vi "EndevoGOOP400Provider_Configuration.vi"(1 "ClassRef/ClassPath(If empty Configuration default will be modified)":variant, 5 "Error In":errorcluster) -> (15 "SelectedWireStyleIndex":i32, 19 "Error Out":errorcluster)   [LabVIEW 2020]
uses:
  Common/LvIcon_class/GDSLvIcon_ColorControl.ctl
  SubVIs/GOOP_WirePattern.ctl
  Common/ScriptingFunctions/Scripting_ConnectorPanePatternType.ctl
  Provider_BaseClassInterface/BaseProvider_SubVIs/BaseProvider_WireStyleType.ctl
  SubVIs/GOOP_WireConfigurationType.ctl
  Common/CommonVIs/CommonVIs_ClassIconSelection_Action.ctl
  Provider_BaseClassInterface/BaseProvider_SubVIs/BaseProvider_FileNamingOption.ctl
  GOOP400_SubVIs/GOOP400_Options.ctl
panel:
  in  "File naming option":T1(ring)
  out "IconSelection":picture
  in  "_FlatFolderStructure":bool caption="Use flat folder structure for new classes"
  in  "WireStyleList":T2[](array[typedef])
  in  "DiscardChanges":bool
  in  "Update/AddWireStyle":bool
  in  "DeleteWireStyle":bool
  in  "Down":bool
  in  "Up":bool
  in  "WireStyleName":string caption="Selected Wire Style Name"
  out "ProductPicture":picture
  out "Icon":picture
  in  "_Dice":cluster{"Boolean 2":bool, "Dice 2":bool}
  in  "_DefaultConnectorPanePattern":T3 caption="Default Connector Pane Pattern" items=["4x4x4", "5x6x5", "6x8x6"]
  in  "_HelpDefaultConfiguration":bool
  in  "_Help":bool
  out "_ClassItemIconApperance":string caption="Class Item Icon Appearance"
  out "_WireApperance":string
  in  "_SetToDefaultForAllClasses":bool caption="Set this to default\nfor all future classes"
  in  "_Cancel":bool
  out "_Preview":picture caption="Preview"
  in  "_Icon":u16(ring) caption="Icon" items=["BlueFull", "BlueFrame", "InterfaceBlue", "BlueCircle", "BrownFull", "BrownFrame", "InterfaceBrown", "BrownCircle", "BurgundyFull", "BurgundyFrame", "InterfaceBurgundy", "BurgundyCircle", "CyanFull", "CyanFrame", "InterfaceCyan", "CyanCircle", "DarkBlueFull", "DarkBlueFrame", "InterfaceDarkBlue", "DarkBlueCircle", "ForestGreenFull", "ForestGreenFrame", "InterfaceForestGreen", "ForestGreenCircle", "GrayFull", "GrayFrame", "InterfaceGray", "GrayCircle", "GreenFull", "GreenFrame", "InterfaceGreen", "GreenCircle", "LightGreenFull", "LightGreenFrame", "InterfaceLightGreen", "LightGreenCircle", "LightRedFull", "LightRedFrame", "InterfaceLightRed", "LightRedCircle", "PinkFull", "PinkFrame", "InterfacePink", "PinkCircle", "PurpleFull", "PurpleFrame", "InterfacePurple", "PurpleCircle", "RedFull", "RedFrame", "InterfaceRed", "RedCircle", "YellowFull", "YellowFrame", "InterfaceYellow", "YellowCircle"]
  in  "_TunnelsAndTerminalsColors":T4 caption="Tunnels and \nTerminals Colors"
  in  "_CenterColor2":T4 caption="Pattern Colors"
  in  "_CenterColor1":T4 caption="Pattern Colors"
  in  "_CenterPattern":T5 caption="Center pattern"
  in  "_EdgeColor":T4 caption="Edge color"
  in  "_CenterThickness":T6(ring) caption="Center thickness"
  in  "_EdgeThickness":T7(ring) caption="Edge thickness"
  out "Wire preview":picture
  in  "_Done":bool
  # "Wire Configuration"
  # "Wire Appearance"
  # "GOOP4 Options"
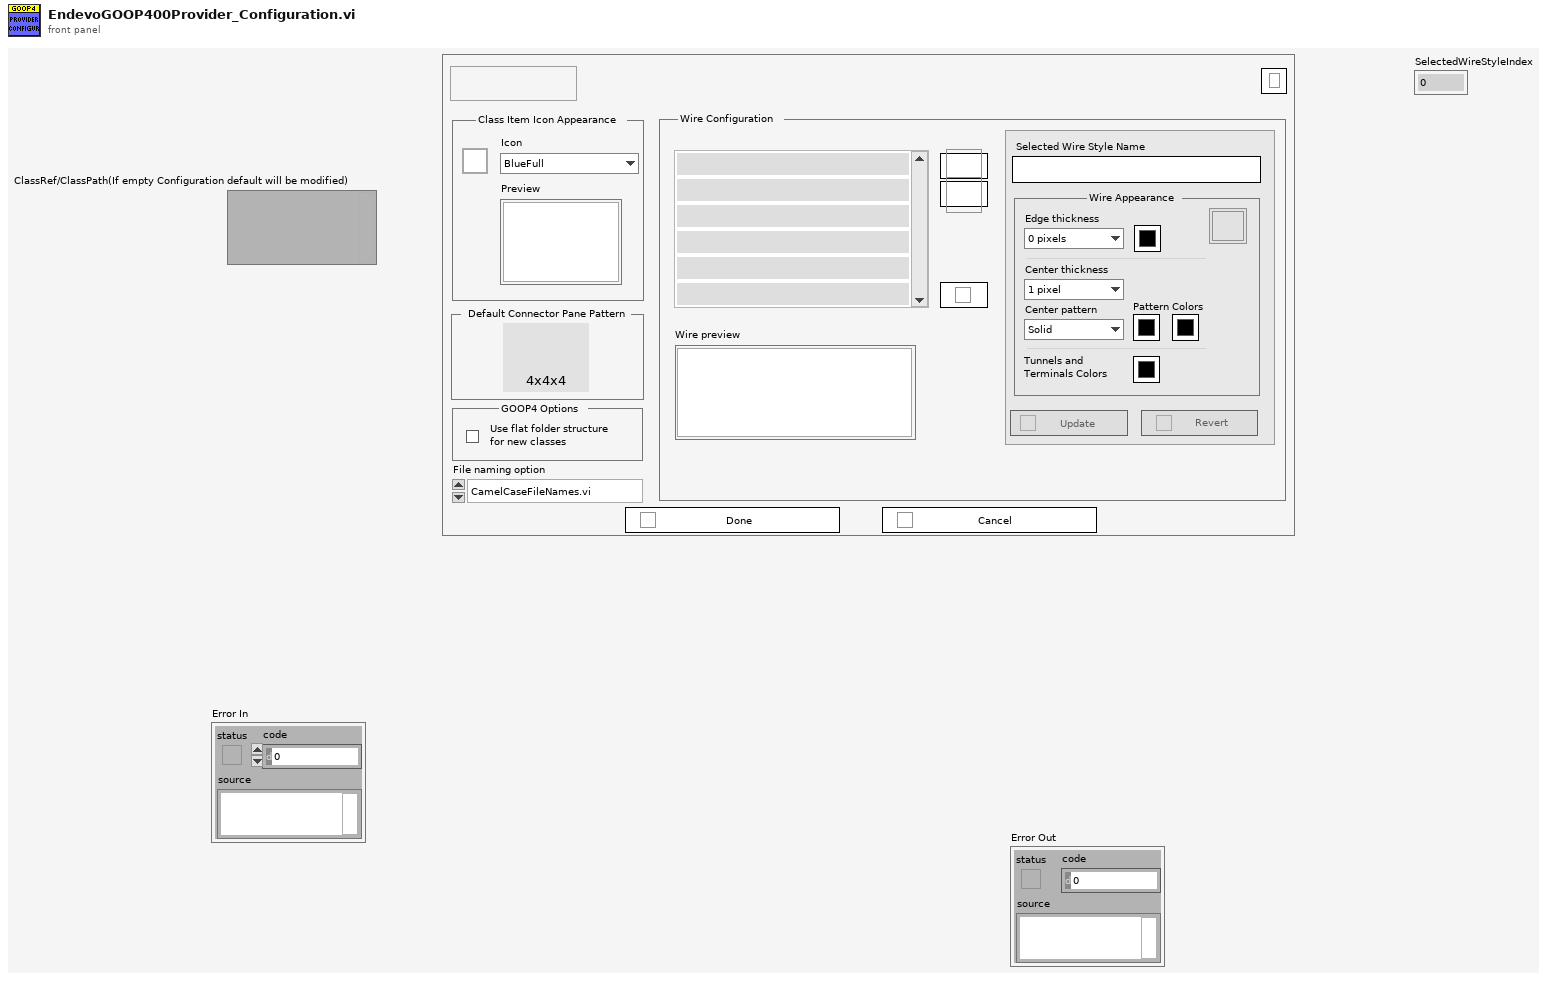
[diagram p1: front panel]
types:
  T1 = enum16{"CamelCaseFileNames.vi", "File Names With Spaces.vi", "File_Names_With_Underscores"}
  T2 = typedef "BaseProvider_WireStyleType.ctl" = cluster{"Boolean":bool, "Wire":picture, "Name":string, "Status":u16}
  T3 = typedef "Scripting_ConnectorPanePatternType.ctl" = u16
  T4 = typedef "GDSLvIcon_ColorControl.ctl" = cluster{"Decal":bool, "Color":u32}
  T5 = typedef "GOOP_WirePattern.ctl" = enum16{"Solid", "Large dash", "Small dash"}
  T6 = enum16{"1 pixel", "2 pixels", "3 pixels", "4 pixels", "5 pixels"}
  T7 = enum16{"0 pixels", "1 pixel", "2 pixels", "3 pixels"}
  T8 = typedef "GOOP_WireConfigurationType.ctl" = cluster{"Edge thickness":i32, "Edge color":u32, "Center thickness":i32, "Center pattern":T5, "CenterColor1":u32, "CenterColor2":u32, "Tunnels and terminals colors":u32}
  T9 = cluster{"FirstTime":bool, "ClassRef":refnum<vi>, "ClassRefCreated":bool, "CurrentWireStyle":T8, "DefaultIndex":i32, "SelectedWireStyleIndex":i32, "StartWireStyleIndex":i32}
  T10 = typedef "GOOP400_Options.ctl" = cluster{"FlatFolderStructure":bool}
  T11 = typedef "BaseProvider_FileNamingOption.ctl" = enum16{"CamelCase", "Space", "Underscore"}
  T12 = typedef "BaseProvider_IniFileSettings.ctl" = cluster{"ClassFolderSuffix":string, "InterfaceFolderSuffix":string, "InterfaceIcon":string, "FileNamingOption":T11, "DynamicDispatchStartValue":bool}
  T13 = typedef "GDSLvCLass_ClassSettingsType.ctl" = cluster{"ClassProviderName":string, "ClassTemplateUsed":string, "ClassTemplateVersion":string, "ClassDescription":string, "PlugIns":T14[], "ConnectorPanePattern":string}
  T14 = typedef "GDSLvClass_PlugIn.ctl" = cluster{"Type":T15, "ID":string, "Version":string, "Path":path, "Name":string, "Data":variant}
  T15 = typedef "GDSLvClass_PlugInTypes.ctl" = enum16{"DesignPattern", "MethodTypes"}
  T16 = cluster{"Foreground Color":u32, "Background Color":u32, "Fill Pattern":cluster{"Row 0":u8, "Row 1":u8, "Row 2":u8, "Row 3":u8, "Row 4":u8, "Row 5":u8, "Row 6":u8, "Row 7":u8}, "Width":i16, "Mode":enum16{"Copy", "Or", "Exclusive Or", "Bit Clear", "Not Copy", "Not Or", "Nor Exclusive Or", "Not Bit Clear"}, "Style":enum32{"Solid", "Dash", "Dot", "Dash Dot", "Dash Dot Dot"}, "Fill Rule":enum32{"Even Odd", "Winding"}, "End Caps":enum32{"Default", "Flat"}}[]
  T17 = enum8{"Enabled", "Disabled", "Disabled and Grayed Out"}
  T18 = typedef "imagedata.ctl" = cluster{"image type":i32, "image depth":i32, "image":u8[], "mask":u8[], "colors":u32[], "Rectangle":cluster{"left":i16, "top":i16, "right":i16, "bottom":i16}}
  T19 = typedef "CommonVIs_ClassIconSelection_Action.ctl" = enum16{"All", "Non Interface", "Only Interface"}
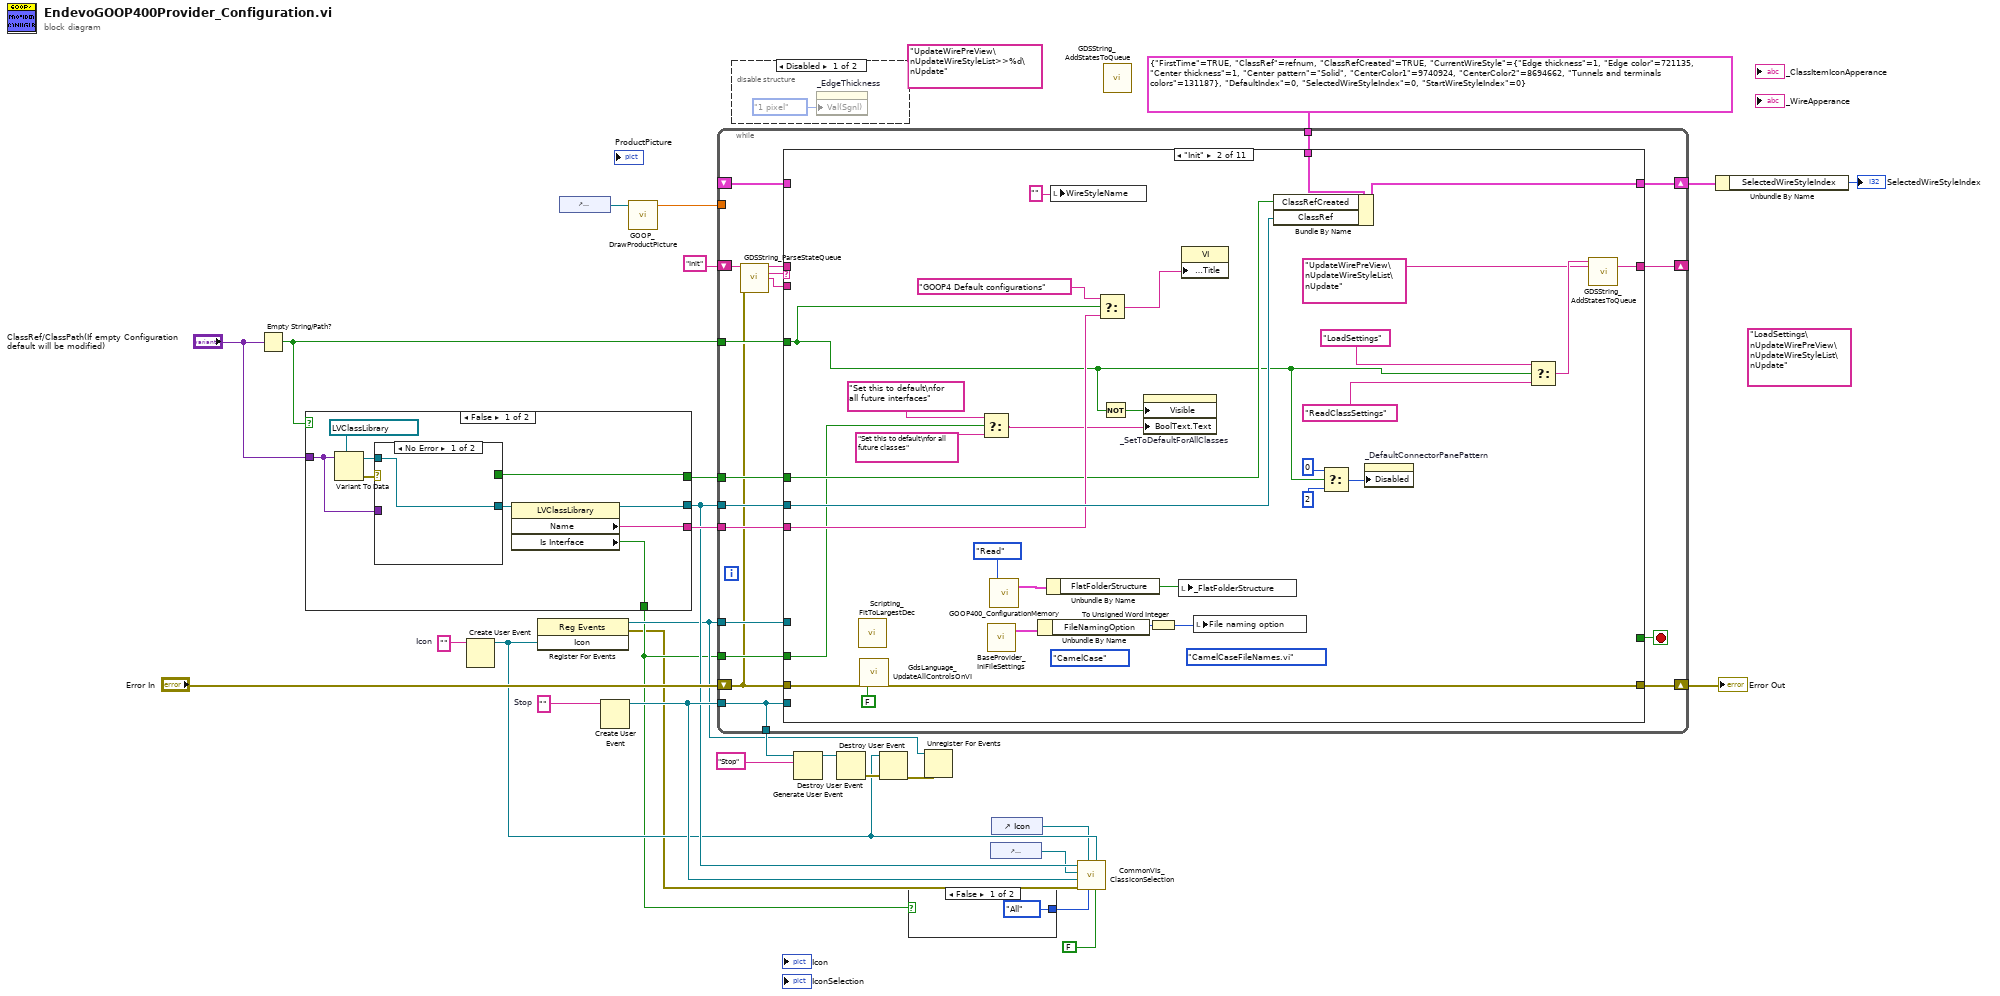
[diagram p0: block diagram]
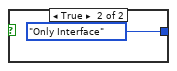
[diagram p2: hidden frame]
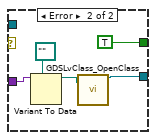
[diagram p4: hidden frame]
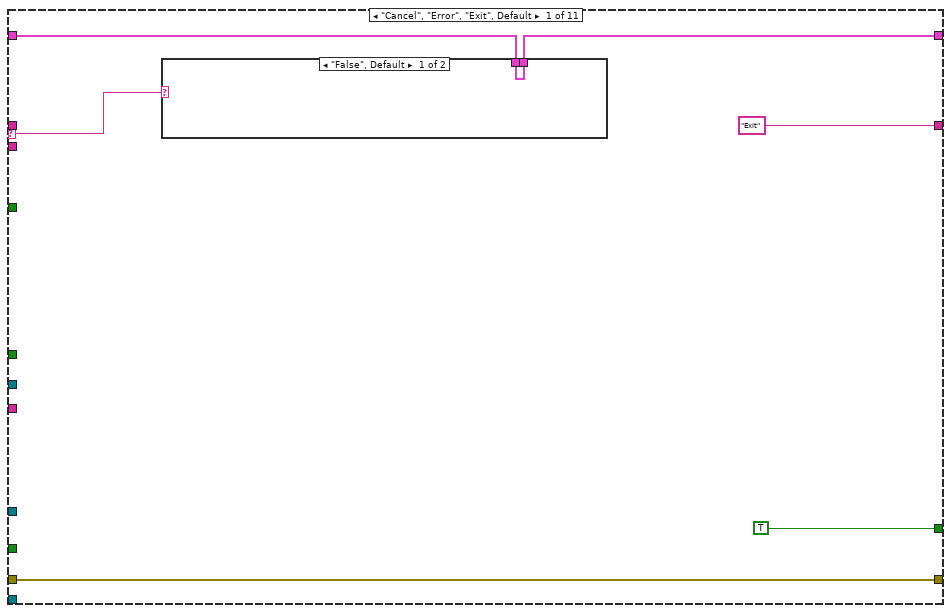
[diagram p6: hidden frame]
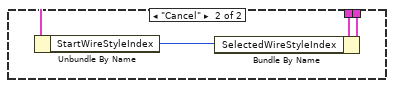
[diagram p7: hidden frame]
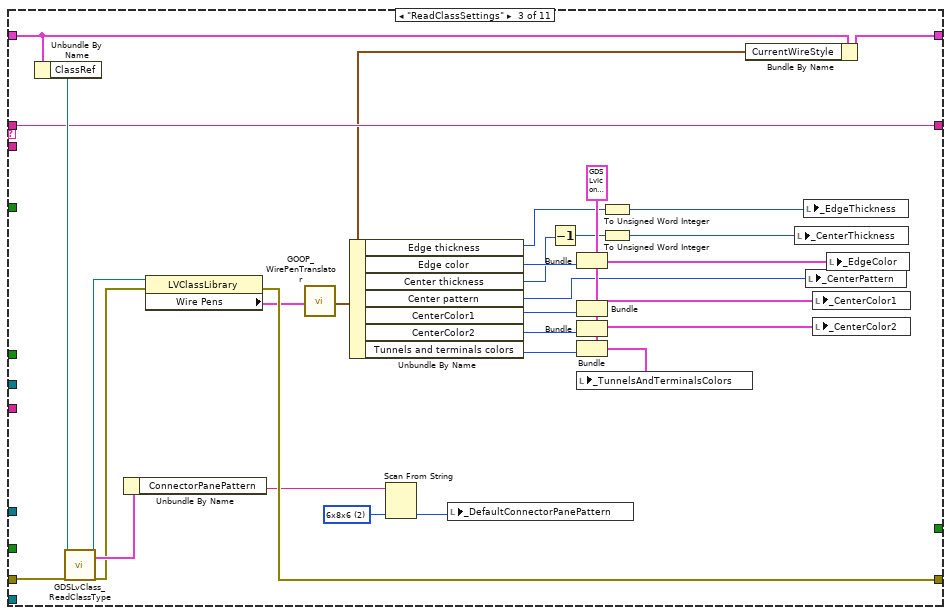
[diagram p8: hidden frame]
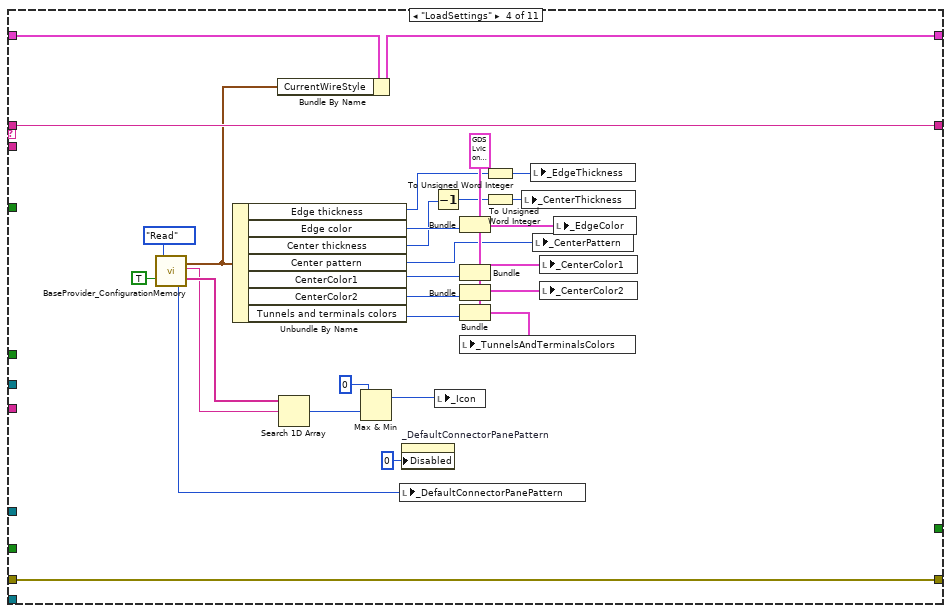
[diagram p9: hidden frame]
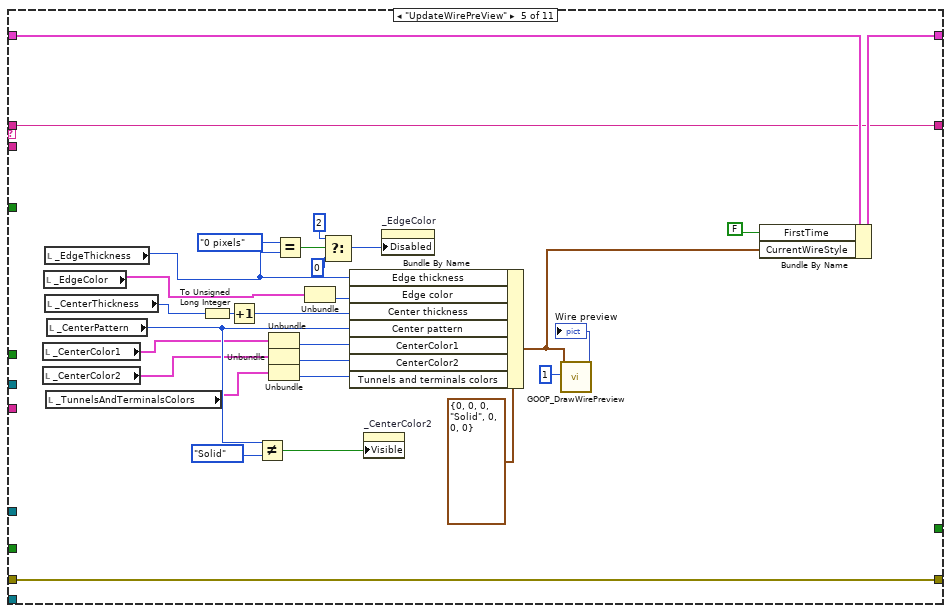
[diagram p10: hidden frame]
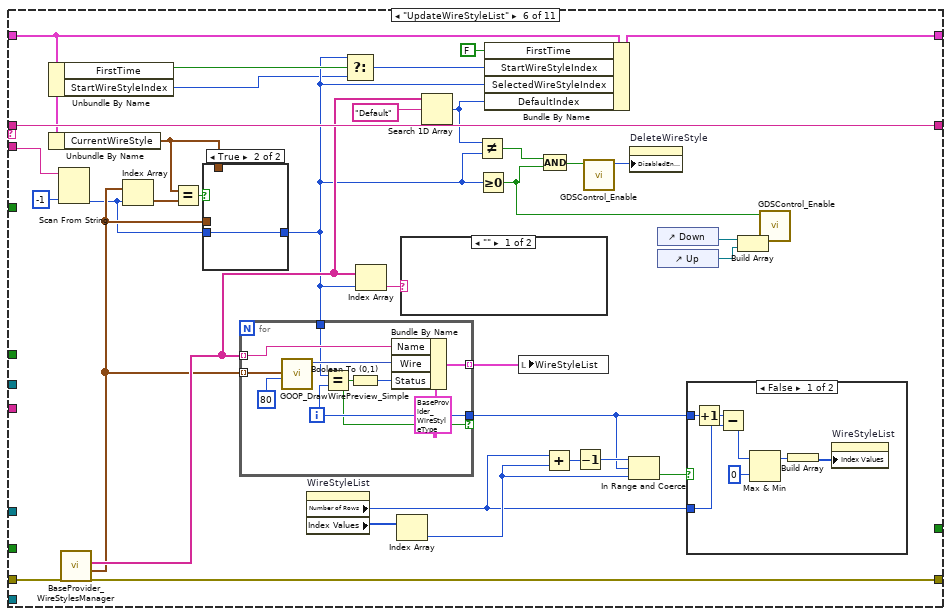
[diagram p11: hidden frame]
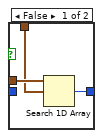
[diagram p12: hidden frame]
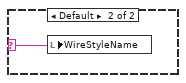
[diagram p14: hidden frame]
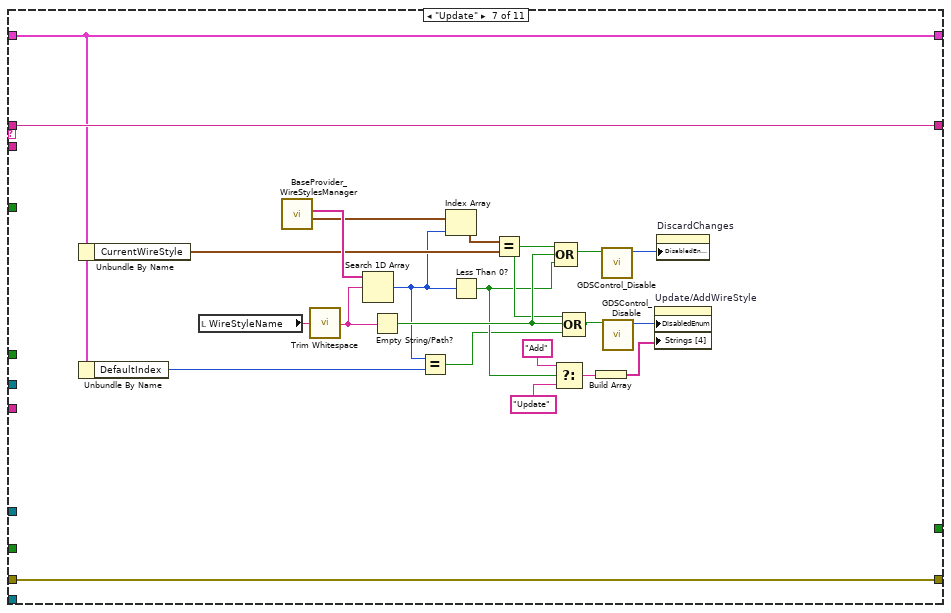
[diagram p15: hidden frame]
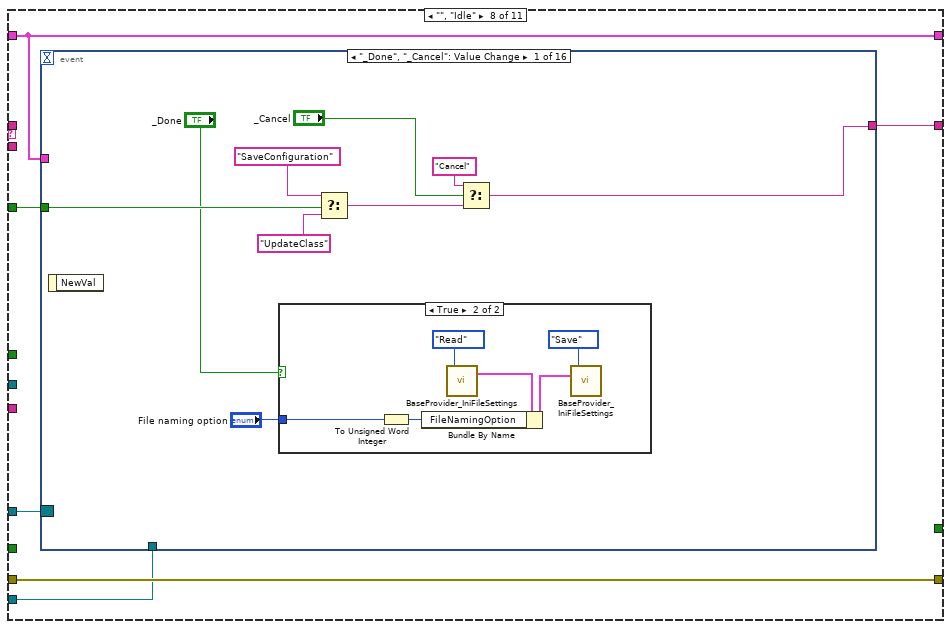
[diagram p16: hidden frame]
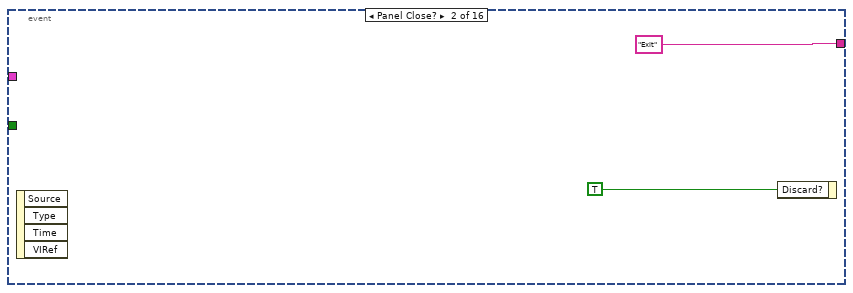
[diagram p18: hidden frame]
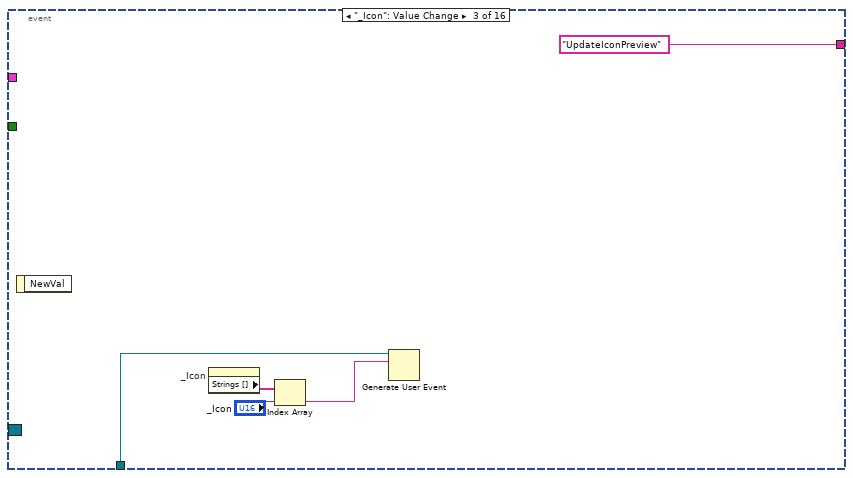
[diagram p19: hidden frame]
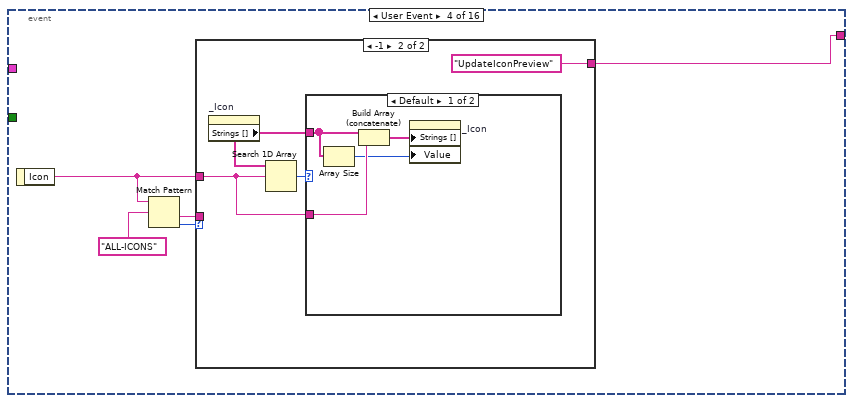
[diagram p20: hidden frame]
diagram:
  (unwired) "LoadSettings\nUpdateWirePreView\nUpdateWireStyleList\nUpdate"
  (unwired) "UpdateWirePreView\nUpdateWireStyleList>>%d\nUpdate"
  w16 = ""  # Icon
  w19 = ""  # Stop
  n1 = Empty String/Path?(string/path="ClassRef/ClassPath(If empty Configuration default will be modified)") -> (empty?=w21:bool)
  n2 = case shown="False" w21 {
    tunnel: "ClassRef/ClassPath(If empty Configuration default will be modified)" -> [w36 _]
    tunnel: [w32 _] -> w17
    tunnel: [w34 _] -> w24
    tunnel: [w31 _] -> w23
    tunnel: [w30 _] -> w11
    frame False {
      n3 = Variant To Data(type=refnum<vi> refnum ("Class Refnum In"), Variant=w36) -> (data=w35:refnum<vi>, error out=w37:errorcluster)  [unwired: 1 in]
      n4 = case shown="No Error" w37 {
        tunnel: w36 -> [_ w44]
        tunnel: [w39 w41] -> w33
        tunnel: w35 -> [w39 _]
        tunnel: [_ TRUE] -> w34
        frame No Error {
        }
        frame Error {
          n5 = Variant To Data(type=path "", Variant=w44) -> (data=w42:path)  [unwired: 1 in, 1 out]
          n6 = call "GDSLvClass_OpenClass.vi"("ClassToOpen"=w42) -> ("LVClass.Open"=w41:refnum<vi>)  [unwired: 17 in, 1 out]
        }
      }
      n7 = property class="LVClassLibrary"(reference=w33) -> (reference out=w32:refnum<vi>, "Name"=w31:string, "Is Interface"=w30:bool)  [unwired: 1 in, 1 out]
    }
    frame True {
    }
  }
  n8 = Create User Event(user event datatype=w16) -> (user event=w12:refnum<user-event>)  [unwired: 1 in, 1 out]
  n9 = register-events(w12) -> (reference out=w15:refnum<event-registration>, error out=w10:errorcluster)  [unwired: 2 in]
  n10 = control-ref of="ProductPicture"() -> (w9:refnum<vi>)
  n11 = Create User Event(user event datatype=w19) -> (user event=w20:refnum<user-event>)  [unwired: 1 in, 1 out]
  n12 = call "GOOP_DrawProductPicture.vi"("ProductPictureControl"=w9) -> ("Zoom Factor"=w8:sgl)  [unwired: 10 in]
  n13 = while {
    shift-right: [w62] -> w27
    shift-left: "Error In" -> [w51]
    shift-right: [w47] -> _
    shift-left: "Init" -> [w52]
    shift-right: [w61] -> w6
    shift-left: _ -> [w60]
    tunnel: w20 -> [w55]
    tunnel: [w55] -> w25
    tunnel: w21 -> [w59]
    tunnel: w17 -> [w58]
    tunnel: w24 -> [w57]
    tunnel: w23 -> [w56]
    tunnel: w15 -> [w54]
    tunnel: w11 -> [w53]
    tunnel: w8 -> [_]
    tunnel: T9 {"FirstTime"=TRUE, "ClassRef"=refnum, "ClassRefCreated"=TRUE, "CurrentWireStyle"={"Edge thickness"=1, "Edge color"=721135, "Center thickness"=1, "Center pattern"=enum."Solid", "CenterColor1"=9740924, "CenterColor2"=8694662, "Tunnels and terminals colors"=131187}, "DefaultIndex"=0, "SelectedWireStyleIndex"=0, "StartWireStyleIndex"=0} -> [w45]
    stop <- w46 stop-if-true
    n14 = call "GDSString_ParseStateQueue.vi"("State Queue"=w52, "Error In (no error)"=w51) -> ("Remaining States"=w49:string, "Current State"=w50:string, "Arguments"=w48:string)  [unwired: 9 in, 2 out]
    n15 = case shown="\"Init\"" w50 {
      selector: w50 -> [w63 _ _ _ _ _ _ _ _ _ _]
      tunnel: w51 -> [w68 w98 w114 w146 w168 w226 w261 w276 w436 w490 w515]
      tunnel: [w68 w97 w131 w146 w168 w223 w261 w276 w442 w490 w515] -> w62
      tunnel: ["Exit" w82 w107 w136 w162 w225 w271 w277 w469 "Idle" "Exit"] -> w47
      tunnel: [w65 w100 w106 w134 w167 w212 w252 w272 w464 w491 w499] -> w61
      tunnel: w60 -> [w64 _ w132 w133 w163 w195 w252 w272 w464 w491 w513]
      tunnel: w59 -> [_ w88 _ _ _ _ _ w275 _ _ _]
      tunnel: w58 -> [_ w95 _ _ _ _ _ _ _ _ _]
      tunnel: w57 -> [_ w93 _ _ _ _ _ _ _ _ _]
      tunnel: w56 -> [_ w94 _ _ _ _ _ _ _ _ _]
      tunnel: w55 -> [_ _ _ _ _ _ _ w273 _ _ _]
      tunnel: w54 -> [_ _ _ _ _ _ _ w274 _ _ _]
      tunnel: w53 -> [_ w92 _ _ _ _ _ _ _ _ w510]
      tunnel: w49 -> [_ _ w107 w136 w162 w225 w271 _ _ _ _]
      tunnel: w48 -> [_ _ _ _ _ w202 _ _ _ _ _]
      tunnel: [TRUE _ _ _ _ _ _ _ _ _ _] -> w46
      tunnel: w45 -> [_ w81 _ _ _ _ _ _ _ _ _]
      frame "Cancel", "Error", "Exit", Default {
        n16 = case shown="\"False\", Default" w63 {
          tunnel: [w69 w72] -> w65
          tunnel: w64 -> [w69 w71]
          frame "False", Default {
          }
          frame "Cancel" {
            n17 = Unbundle By Name(w71) -> ("StartWireStyleIndex"=w70:i32)
            n18 = Bundle By Name(cluster=w71, "SelectedWireStyleIndex"=w70) -> (w72:T9)
          }
        }
      }
      frame "Init" {
        (unwired) T1."CamelCaseFileNames.vi" ("File naming option")
        (unwired) BaseProvider_FileNamingOption."CamelCase" ("FileNamingOption")
        n19 = call "Scripting_FitToLargestDec.vi"() -> ()  [unwired: 6 in, 2 out]
        n20 = call "GdsLanguage_UpdateAllControlsOnVI.vi"("error in (no error)"=w98, "CreateLanguageFile(Use this to create a languageFile)"=FALSE) -> ("error out"=w97:errorcluster)  [unwired: 16 in, 1 out]
        n21 = Select(t="Set this to default\nfor all future interfaces", s=w92, f="Set this to default\nfor all future classes") -> (s? t:f=w89:string)
        n22 = call "BaseProvider_IniFileSettings.vi"() -> ("IniFileSettings"=w75:T12)  [unwired: 18 in, 1 out]
        n23 = call "GOOP400_ConfigurationMemory.vi"("Action"=enum16{"Read", "Load", "Save"}."Read") -> ("OptionsOut"=w78:T10)  [unwired: 17 in, 1 out]
        n24 = Unbundle By Name(w75) -> ("FileNamingOption"=w74:T11)
        n25 = Unbundle By Name(w78) -> ("FlatFolderStructure"=w76:bool)
        n26 = local write "WireStyleName"("" ("WireStyleName")) -> ()
        n27 = Select(t="GOOP4 Default configurations", s=w88, f=w94) -> (s? t:f=w79:string)
        n28 = Not(x=w88) -> (.not. x?=w99:bool)
        n29 = property on="_SetToDefaultForAllClasses" class="Bool (strict)"("Visible"=w99, "BoolText.Text"=w89) -> ()  [unwired: 2 in, 2 out]
        n30 = To Unsigned Word Integer(number=w74) -> (unsigned 16bit integer=w73:u16)
        n31 = local write "_FlatFolderStructure"(w76) -> ()
        n32 = property class="VI"("Front Panel.Title"=w79) -> ()  [unwired: 2 in, 2 out]
        n33 = local write "File naming option"(w73) -> ()
        n34 = Bundle By Name(cluster=w81, "ClassRefCreated"=w93, "ClassRef"=w95) -> (w100:T9)
        n35 = Select(t=u8 0 ("Disabled"), s=w88, f=u8 2 ("Disabled")) -> (s? t:f=w86:u8)
        n36 = property on="_DefaultConnectorPanePattern" class="Ring (strict)"("Disabled"=w86) -> ()  [unwired: 2 in, 2 out]
        n37 = Select(t="LoadSettings", s=w88, f="ReadClassSettings") -> (s? t:f=w84:string)
        n38 = call "GDSString_AddStatesToQueue.vi"("State(s) in Front (\"\")"=w84, "State(s) in (\"\")"="UpdateWirePreView\nUpdateWireStyleList\nUpdate") -> ("States Out"=w82:string)  [unwired: 13 in]
      }
      frame "ReadClassSettings" {
        w111 = T3 2 items=["4x4x4", "5x6x5", "6x8x6"] ("Pattern")
        w124 = T4 {"Decal"=FALSE, "Color"=11184810} ("Edge color")
        n39 = Unbundle By Name(w132) -> ("ClassRef"=w113:refnum<vi>)
        n40 = call "GDSLvClass_ReadClassType.vi"("Class Refnum In"=w113, "error in (no error)"=w114) -> ("Class Refnum Out"=w108:refnum<vi>, "ClassSettings"=w112:T13, "error out"=w104:errorcluster)  [unwired: 15 in]
        n41 = Unbundle By Name(w112) -> ("ConnectorPanePattern"=w110:string)
        n42 = property class="LVClassLibrary"(reference=w108, error in=w104) -> (error out=w131:errorcluster, "Wire Pens"=w130:T16)  [unwired: 1 out]
        n43 = call "GOOP_WirePenTranslator.vi"("WirePensIn"=w130) -> ("WireConfigurationOut"=w105:T8)  [unwired: 17 in, 1 out]
        n44 = Unbundle By Name(w105) -> ("Edge thickness"=w116:i32, "Edge color"=w129:u32, "Center thickness"=w119:i32, "Center pattern"=w120:T5, "CenterColor1"=w128:u32, "CenterColor2"=w127:u32, "Tunnels and terminals colors"=w126:u32)
        n45 = Scan From String(input string=w110, default 1=w111) -> (output 1=w109:T3)  [unwired: 3 in, 3 out]
        n46 = local write "_DefaultConnectorPanePattern"(w109) -> ()
        n47 = Decrement(x=w119) -> (x-1=w118:i32)
        n48 = Bundle(cluster=w124, "Color"=w129) -> (w121:T4)  [unwired: 1 in]
        n49 = Bundle(cluster=w124, "Color"=w128) -> (w122:T4)  [unwired: 1 in]
        n50 = Bundle(cluster=w124, "Color"=w127) -> (w123:T4)  [unwired: 1 in]
        n51 = Bundle(cluster=w124, "Color"=w126) -> (w125:T4)  [unwired: 1 in]
        n52 = local write "_TunnelsAndTerminalsColors"(w125) -> ()
        n53 = To Unsigned Word Integer(number=w116) -> (unsigned 16bit integer=w115:u16)
        n54 = To Unsigned Word Integer(number=w118) -> (unsigned 16bit integer=w117:u16)
        n55 = Bundle By Name(cluster=w132, "CurrentWireStyle"=w105) -> (w106:T9)
        n56 = local write "_CenterThickness"(w117) -> ()
        n57 = local write "_EdgeThickness"(w115) -> ()
        n58 = local write "_CenterPattern"(w120) -> ()
        n59 = local write "_CenterColor1"(w122) -> ()
        n60 = local write "_CenterColor2"(w123) -> ()
        n61 = local write "_EdgeColor"(w121) -> ()
      }
      frame "LoadSettings" {
        w156 = T4 {"Decal"=FALSE, "Color"=11184810} ("Edge color")
        n62 = call "BaseProvider_ConfigurationMemory.vi"("Filter_Icons"=TRUE, "Action"=enum16{"Read", "Load", "Save"}."Read") -> ("PatternOut"=w139:T3, "WireConfigurationOut"=w135:T8, "IconOut"=w143:string, "ClassItemIconNames"=w144:string[])  [unwired: 11 in, 3 out]
        n63 = Unbundle By Name(w135) -> ("Edge thickness"=w148:i32, "Edge color"=w161:u32, "Center thickness"=w151:i32, "Center pattern"=w152:T5, "CenterColor1"=w160:u32, "CenterColor2"=w159:u32, "Tunnels and terminals colors"=w158:u32)
        n64 = Bundle By Name(cluster=w133, "CurrentWireStyle"=w135) -> (w134:T9)
        n65 = Search 1D Array(1D array=w144, element=w143) -> (index of element=w141:i32)  [unwired: 1 in]
        n66 = Max & Min(x=0, y=w141) -> (max(x,y)=w140:i32)  [unwired: 1 out]
        n67 = local write "_DefaultConnectorPanePattern"(w139) -> ()
        n68 = property on="_DefaultConnectorPanePattern" class="Ring (strict)"("Disabled"=u8 0) -> ()  [unwired: 2 in, 2 out]
        n69 = Decrement(x=w151) -> (x-1=w150:i32)
        n70 = local write "_Icon"(w140) -> ()
        n71 = Bundle(cluster=w156, "Color"=w161) -> (w153:T4)  [unwired: 1 in]
        n72 = Bundle(cluster=w156, "Color"=w160) -> (w154:T4)  [unwired: 1 in]
        n73 = Bundle(cluster=w156, "Color"=w159) -> (w155:T4)  [unwired: 1 in]
        n74 = Bundle(cluster=w156, "Color"=w158) -> (w157:T4)  [unwired: 1 in]
        n75 = local write "_TunnelsAndTerminalsColors"(w157) -> ()
        n76 = To Unsigned Word Integer(number=w148) -> (unsigned 16bit integer=w147:u16)
        n77 = To Unsigned Word Integer(number=w150) -> (unsigned 16bit integer=w149:u16)
        n78 = local write "_CenterThickness"(w149) -> ()
        n79 = local write "_EdgeThickness"(w147) -> ()
        n80 = local write "_CenterPattern"(w152) -> ()
        n81 = local write "_CenterColor1"(w154) -> ()
        n82 = local write "_CenterColor2"(w155) -> ()
        n83 = local write "_EdgeColor"(w153) -> ()
      }
      frame "UpdateWirePreView" {
        n84 = local read "_CenterColor1"() -> (w171:T4)
        n85 = local read "_CenterColor2"() -> (w170:T4)
        n86 = local read "_EdgeColor"() -> (w174:T4)
        n87 = local read "_EdgeThickness"() -> (w175:T7)
        n88 = local read "_CenterThickness"() -> (w173:T6)
        n89 = local read "_TunnelsAndTerminalsColors"() -> (w169:T4)
        n90 = local read "_CenterPattern"() -> (w172:T5)
        n91 = To Unsigned Long Integer(number=w173) -> (unsigned 32bit integer=w190:u32)
        n92 = Increment(x=w190) -> (x+1=w183:u32)
        n93 = Not Equal?(x=w172, y=GOOP_WirePattern."Solid") -> (x != y?=w165:bool)
        n94 = Unbundle(w171) -> ("Color"=w181:u32)  [unwired: 1 out]
        n95 = Unbundle(w170) -> ("Color"=w182:u32)  [unwired: 1 out]
        n96 = Unbundle(w169) -> ("Color"=w179:u32)  [unwired: 1 out]
        n97 = Equal?(x=T7."0 pixels", y=w175) -> (x = y?=w185:bool)
        n98 = Unbundle(w174) -> ("Color"=w180:u32)  [unwired: 1 out]
        n99 = Select(t=u8 2 ("Disabled"), s=w185, f=u8 0) -> (s? t:f=w187:u8)
        n100 = Bundle By Name(cluster=T8 {"Edge thickness"=0, "Edge color"=0, "Center thickness"=0, "Center pattern"=enum."Solid", "CenterColor1"=0, "CenterColor2"=0, "Tunnels and terminals colors"=0} ("WireConfiguration"), "Edge thickness"=w175, "Edge color"=w180, "Center thickness"=w183, "Center pattern"=w172, "CenterColor1"=w181, "CenterColor2"=w182, "Tunnels and terminals colors"=w179) -> (w164:T8)
        n101 = property on="_CenterColor2" class="Clust (strict)"("Visible"=w165) -> ()  [unwired: 2 in, 2 out]
        n102 = property on="_EdgeColor" class="Clust (strict)"("Disabled"=w187) -> ()  [unwired: 2 in, 2 out]
        n103 = call "GOOP_DrawWirePreview.vi"("WireConfiguration"=w164, "Zoom"=1) -> ("Picture"=→"Wire preview":picture)  [unwired: 16 in, 1 out]
        n104 = Bundle By Name(cluster=w163, "FirstTime"=FALSE, "CurrentWireStyle"=w164) -> (w167:T9)
      }
      frame "UpdateWireStyleList" {
        n105 = Unbundle By Name(w195) -> ("FirstTime"=w194:bool, "StartWireStyleIndex"=w191:i32)
        n106 = Unbundle By Name(w195) -> ("CurrentWireStyle"=w200:T8)
        n107 = Scan From String(input string=w202, default 1=-1 ("default value 1")) -> (output 1=w197:i32)  [unwired: 3 in, 3 out]
        n108 = call "BaseProvider_WireStylesManager.vi"("error in (no error)"=w226) -> ("error out"=w223:errorcluster, "AllWireConfigurations"=w203:T8[], "AllWireConfigurations(Names)"=w214:string[])  [unwired: 7 in, 1 out]
        n109 = Index Array(array=w203, index=w197) -> (element=w199:T8)
        n110 = Equal?(x=w200, y=w199) -> (x = y?=w198:bool)
        n111 = case shown="True" w198 {
          tunnel: [w229 w230] -> w193
          tunnel: w203 -> [w228 _]
          tunnel: w200 -> [w227 _]
          tunnel: w197 -> [_ w230]
          frame False {
            n112 = Search 1D Array(1D array=w228, element=w227) -> (index of element=w229:i32)  [unwired: 1 in]
          }
          frame True {
          }
        }
        n113 = for {
          tunnel: w214 -> [w244] mode=indexing
          tunnel: w203 -> [w247] mode=indexing
          tunnel: [w243] -> w224 mode=indexing
          tunnel: w193 -> [w242]
          tunnel: [w240] -> w216 if=w239
          i -> [w240]
          n114 = call "GOOP_DrawWirePreview_Simple.vi"("WireLength(100px)"=i16 80, "WireConfiguration"=w247) -> ("WirePictureOut"=w245:picture)  [unwired: 5 in, 4 out]
          n115 = Equal?(x=w242, y=w240) -> (x = y?=w239:bool)
          n116 = Boolean To (0,1)(Boolean=w239) -> (0, 1=w241:i16)
          n117 = Bundle By Name(cluster=T2 {"Boolean"=FALSE, "Wire"=bytes[0], "Name"="", "Status"=0} ("Cluster 2"), "Name"=w244, "Wire"=w245, "Status"=w241) -> (w243:T2)
        }
        n118 = property on="WireStyleList" class="Arr (strict)"() -> ("Number of Rows"=w215:u32, "Index Values"=w221:u32[])  [unwired: 2 in, 2 out]
        n119 = Select(t=w193, s=w194, f=w191) -> (s? t:f=w192:i32)
        n120 = Index Array(array=w214, index=w193) -> (element=w222:string)
        n121 = Index Array(array=w221) -> (element=w220:u32)  [unwired: 1 in]
        n122 = case shown="\"\"" w222 {
          selector: w222 -> [_ w238]
          frame "" {
          }
          frame Default {
            n123 = local write "WireStyleName"(w238) -> ()
          }
        }
        n124 = Search 1D Array(1D array=w214, element="Default") -> (index of element=w211:i32)  [unwired: 1 in]
        n125 = Not Equal?(x=w211, y=w193) -> (x != y?=w210:bool)
        n126 = Greater Or Equal To 0?(x=w193) -> (x >= 0?=w207:bool)
        n127 = Bundle By Name(cluster=w195, "FirstTime"=FALSE, "StartWireStyleIndex"=w192, "SelectedWireStyleIndex"=w193, "DefaultIndex"=w211) -> (w212:T9)
        n128 = local write "WireStyleList"(w224) -> ()
        n129 = Compound Arithmetic op=AND(w210, w207) -> (w209:bool)
        n130 = Add(x=w215, y=w220) -> (x+y=w219:u32)
        n131 = Decrement(x=w219) -> (x-1=w218:u32)
        n132 = call "GDSControl_Enable.vi"("Enable(True)"=w209) -> ("Enable Property"=w208:T17)  [unwired: 10 in]
        n133 = In Range and Coerce(upper limit=w218, x=w216, lower limit=w220) -> (In Range?=w217:bool)  [unwired: 1 out]
        n134 = property on="DeleteWireStyle" class="Bool"("DisabledEnum"=w208) -> ()  [unwired: 2 in, 2 out]
        n135 = control-ref of="Down"() -> (w206:refnum<vi>)
        n136 = control-ref of="Up"() -> (w205:refnum<vi>)
        n137 = case shown="False" w217 {
          tunnel: w216 -> [w236 _]
          tunnel: w215 -> [w235 _]
          frame False {
            n138 = Increment(x=w236) -> (x+1=w231:i32)
            n139 = Subtract(x=w231, y=w235) -> (x-y=w234:u32)
            n140 = Max & Min(x=w234, y=u32 0) -> (max(x,y)=w232:u32)  [unwired: 1 out]
            n141 = Build Array(w232) -> (w237:u32[])
            n142 = property on="WireStyleList" class="Arr (strict)"("Index Values"=w237) -> ()  [unwired: 2 in, 2 out]
          }
          frame True {
          }
        }
        n143 = Build Array(w206, w205) -> (w204:refnum<vi>[])
        n144 = call "GDSControl_Enable.vi"("ManyControls"=w204, "Enable(True)"=w207) -> ()  [unwired: 9 in, 1 out]
      }
      frame "Update" {
        n145 = Unbundle By Name(w252) -> ("CurrentWireStyle"=w265:T8)
        n146 = Unbundle By Name(w252) -> ("DefaultIndex"=w250:i32)
        n147 = local read "WireStyleName"() -> (w270:string)
        n148 = call "BaseProvider_WireStylesManager.vi"() -> ("AllWireConfigurations"=w266:T8[], "AllWireConfigurations(Names)"=w268:string[])  [unwired: 8 in, 2 out]
        n149 = call <vilib>:"Trim Whitespace.vi"("string"=w270) -> ("trimmed string"=w267:string)  [unwired: 1 in]
        n150 = Search 1D Array(1D array=w268, element=w267) -> (index of element=w251:i32)  [unwired: 1 in]
        n151 = Empty String/Path?(string/path=w267) -> (empty?=w260:bool)
        n152 = Equal?(x=w251, y=w250) -> (x = y?=w249:bool)
        n153 = Index Array(array=w266, index=w251) -> (element=w264:T8)
        n154 = Less Than 0?(x=w251) -> (x < 0?=w257:bool)
        n155 = Equal?(x=w264, y=w265) -> (x = y?=w258:bool)
        n156 = Select(t="Add", s=w257, f="Update") -> (s? t:f=w254:string)
        n157 = Compound Arithmetic op=OR(w258, w260, w257) -> (w263:bool)
        n158 = Compound Arithmetic op=OR(w258, w260, w249) -> (w259:bool)
        n159 = Build Array(w254) -> (w253:string[])
        n160 = call "GDSControl_Disable.vi"("Disasble(True)"=w263) -> ("Enable Property"=w262:T17)  [unwired: 10 in]
        n161 = call "GDSControl_Disable.vi"("Disasble(True)"=w259) -> ("Enable Property"=w269:T17)  [unwired: 10 in]
        n162 = property on="Update/AddWireStyle" class="Bool"("DisabledEnum"=w269, "Strings [4]"=w253) -> ()  [unwired: 2 in, 2 out]
        n163 = property on="DiscardChanges" class="Bool"("DisabledEnum"=w262) -> ()  [unwired: 2 in, 2 out]
      }
      frame "", "Idle" {
        n164 = event shown="[0] \"_Done\", \"_Cancel\": Value Change" {
          selector: w274 -> [_ _ _ _ _ _ _ _ _ _ _ _ _ _ _ _]
          dyn-events: _ -> [_ _ _ _ _ _ _ _ _ _ _ _ _ _ _ _]
          timeout: _ -> [_ _ _ _ _ _ _ _ _ _ _ _ _ _ _ _]
          tunnel: [w282 "Exit" "UpdateIconPreview" w300 "UpdateWirePreView\nUpdate" "Idle" "UpdateWirePreView\nUpdate" w331 "Update" w362 "UpdateWirePreView\nUpdateWireStyleList\nUpdate" "UpdateWirePreView\nUpdateWireStyleList\nUpdate" w407 "Idle" "Idle" "Idle"] -> w277
          tunnel: w275 -> [w280 _ _ _ _ _ _ _ _ _ _ _ _ _ _ _]
          tunnel: w273 -> [_ _ w297 _ _ _ _ _ _ _ _ _ _ _ _ _]
          tunnel: w272 -> [_ _ _ _ _ _ _ _ _ _ _ w402 w416 _ _ _]
          event "_Done", "_Cancel": Value Change {
            n165 = event-data() -> ()  [unwired: 1 in, 1 out]
            n166 = case shown="True" "_Done" {
              tunnel: "File naming option" -> [_ w287]
              frame False {
              }
              frame True {
                n167 = To Unsigned Word Integer(number=w287) -> (unsigned 16bit integer=w288:u16)
                n168 = call "BaseProvider_IniFileSettings.vi"("Action"=enum16{"Read", "Load", "Save"}."Read") -> ("IniFileSettings"=w292:T12)  [unwired: 17 in, 1 out]
                n169 = Bundle By Name(cluster=w292, "FileNamingOption"=w288) -> (w289:T12)
                n170 = call "BaseProvider_IniFileSettings.vi"("IniFileSettings"=w289, "Action"=enum16{"Read", "Load", "Save"}."Save") -> ()  [unwired: 16 in, 2 out]
              }
            }
            n171 = Select(t="SaveConfiguration", s=w280, f="UpdateClass") -> (s? t:f=w283:string)
            n172 = Select(t="Cancel", s="_Cancel", f=w283) -> (s? t:f=w282:string)
          }
          event Panel Close? {
            n173 = event-data() -> ()  [unwired: 1 in, 4 out]
            n174 = event-data("Discard?"=TRUE) -> ()  [unwired: 1 in, 1 out]
          }
          event "_Icon": Value Change {
            n175 = event-data() -> ()  [unwired: 1 in, 1 out]
            n176 = property on="_Icon" class="Ring (strict)"() -> ("Strings []"=w298:string[])  [unwired: 2 in, 2 out]
            n177 = Index Array(array=w298, index="_Icon") -> (element=w296:string)
            n178 = Generate User Event(user event=w297, event data cluster=w296) -> ()  [unwired: 2 in, 2 out]
          }
          event User Event {
            n179 = event-data() -> ("Icon"=w304:string)  [unwired: 1 in]
            n180 = Match Pattern(string=w304, regular expression="ALL-ICONS" ("string")) -> (after substring=w301:string, offset past match=w302:i32)  [unwired: 1 in, 2 out]
            n181 = case shown="-1" w302 {
              tunnel: w304 -> [_ w310]
              tunnel: w301 -> [w306 _]
              tunnel: ["Idle" "UpdateIconPreview"] -> w300
              frame 0, Default {
                n182 = Spreadsheet String To Array(format string="%s", spreadsheet string=w306, array type (2D Dbl)=string[] []) -> (array=w309:string[])  [unwired: 1 in]
                n183 = property on="_Icon" class="Ring (strict)"("Strings []"=w309) -> ()  [unwired: 2 in, 2 out]
              }
              frame -1 {
                n184 = property on="_Icon" class="Ring (strict)"() -> ("Strings []"=w311:string[])  [unwired: 2 in, 2 out]
                n185 = Search 1D Array(1D array=w311, element=w310) -> (index of element=w313:i32)  [unwired: 1 in]
                n186 = case shown="Default" w313 {
                  selector: w313 -> [_ w318]
                  tunnel: w311 -> [w315 _]
                  tunnel: w310 -> [w316 _]
                  frame Default {
                    n187 = Array Size(array=w315) -> (size(s)=w314:i32)
                    n188 = Build Array (concatenate)(w315, w316) -> (w317:string[])
                    n189 = property on="_Icon" class="Ring (strict)"("Strings []"=w317, "Value"=w314) -> ()  [unwired: 2 in, 2 out]
                  }
                  frame 0.. {
                    n190 = local write "_Icon"(w318) -> ()
                  }
                }
              }
            }
          }
          event "_EdgeThickness", "_CenterThickness": Value Change {
            n191 = event-data() -> ()  [unwired: 1 in, 1 out]
          }
          event "_Help": Value Change {
            n192 = event-data() -> ()  [unwired: 1 in, 1 out]
            n193 = call "GOOP_HelpMain.vi"() -> ()  [unwired: 12 in]
          }
          event "_Dice": Value Change {
            n194 = event-data() -> ()  [unwired: 1 in, 1 out]
            n195 = control-ref of="_TunnelsAndTerminalsColors"() -> (w328:refnum<vi>)
            n196 = control-ref of="_EdgeColor"() -> (w326:refnum<vi>)
            n197 = control-ref of="_CenterColor1"() -> (w323:refnum<vi>)
            n198 = control-ref of="_CenterColor2"() -> (w322:refnum<vi>)
            n199 = control-ref of="_CenterPattern"() -> (w327:refnum<vi>)
            n200 = control-ref of="_CenterThickness"() -> (w325:refnum<vi>)
            n201 = control-ref of="_EdgeThickness"() -> (w324:refnum<vi>)
            n202 = call "BaseProvider_RandomWireConfig.vi"("EdgeColor"=w326, "_CenterThickness"=w325, "_EdgeThickness"=w324, "_CenterColor2"=w323, "_CenterColor1"=w322, "_CenterPattern"=w327, "_TunnelsAndTerminalsColors"=w328) -> ()  [unwired: 13 in]
            n203 = local write "_Dice"(cluster{"Boolean 2":bool, "Dice":bool} {"Boolean 2"=TRUE, "Dice"=FALSE} ("Dice")) -> ()
          }
          event "WireStyleList": Value Change {
            n204 = event-data() -> ("OldVal"=w330:T2[], "NewVal"=w335:T2[])  [unwired: 1 in, 1 out]
            n205 = for {
              tunnel: w335 -> [w360] mode=indexing
              tunnel: [w359] -> w334 mode=indexing
              n206 = Unbundle By Name(w360) -> ("Boolean"=w359:bool)
            }
            n207 = Search 1D Array(1D array=w334, element=TRUE) -> (index of element=w332:i32)  [unwired: 1 in]
            n208 = case shown="0, Default" w332 {
              selector: w332 -> [w338 _]
              tunnel: [w336 _] -> w331
              tunnel: w330 -> [w341 _]
              frame 0, Default {
                w343 = T4 {"Decal"=FALSE, "Color"=11184810} ("Edge color")
                n209 = call "BaseProvider_WireStylesManager.vi"() -> ("AllWireConfigurations"=w358:T8[], "AllWireConfigurations(Names)"=w340:string[])  [unwired: 8 in, 2 out]
                n210 = local write "WireStyleList"(w341) -> ()
                n211 = Index Array(array=w340, index=w338) -> (element=w339:string)
                n212 = Index Array(array=w358, index=w338) -> (element=w342:T8)
                n213 = local write "WireStyleName"(w339) -> ()
                n214 = Unbundle By Name(w342) -> ("Edge thickness"=w345:i32, "Edge color"=w357:u32, "Center thickness"=w348:i32, "Center pattern"=w349:T5, "CenterColor1"=w356:u32, "CenterColor2"=w355:u32, "Tunnels and terminals colors"=w354:u32)
                n215 = Format Into String(format string="UpdateWirePreView\nUpdateWireStyleList>>%d\nUpdate", w338) -> (resulting string=w336:string)  [unwired: 2 in, 1 out]
                n216 = Decrement(x=w348) -> (x-1=w347:i32)
                n217 = Bundle(cluster=w343, "Color"=w357) -> (w350:T4)  [unwired: 1 in]
                n218 = Bundle(cluster=w343, "Color"=w356) -> (w351:T4)  [unwired: 1 in]
                n219 = Bundle(cluster=w343, "Color"=w355) -> (w352:T4)  [unwired: 1 in]
                n220 = Bundle(cluster=w343, "Color"=w354) -> (w353:T4)  [unwired: 1 in]
                n221 = local write "_TunnelsAndTerminalsColors"(w353) -> ()
                n222 = To Unsigned Word Integer(number=w345) -> (unsigned 16bit integer=w344:u16)
                n223 = To Unsigned Word Integer(number=w347) -> (unsigned 16bit integer=w346:u16)
                n224 = local write "_CenterThickness"(w346) -> ()
                n225 = local write "_EdgeThickness"(w344) -> ()
                n226 = local write "_CenterPattern"(w349) -> ()
                n227 = local write "_CenterColor1"(w351) -> ()
                n228 = local write "_CenterColor2"(w352) -> ()
                n229 = local write "_EdgeColor"(w350) -> ()
              }
              frame -1 {
              }
            }
          }
          event "WireStyleName": Value Change {
            n230 = event-data() -> ()  [unwired: 1 in, 6 out]
          }
          event "DiscardChanges": Value Change {
            n231 = event-data() -> ()  [unwired: 1 in, 1 out]
            n232 = local read "WireStyleName"() -> (w367:string)
            n233 = call "BaseProvider_WireStylesManager.vi"() -> ("AllWireConfigurations"=w364:T8[], "AllWireConfigurations(Names)"=w366:string[])  [unwired: 8 in, 2 out]
            n234 = call <vilib>:"Trim Whitespace.vi"("string"=w367) -> ("trimmed string"=w365:string)  [unwired: 1 in]
            n235 = Search 1D Array(1D array=w366, element=w365) -> (index of element=w363:i32)  [unwired: 1 in]
            n236 = case shown="0, Default" w363 {
              selector: w363 -> [w385 _]
              tunnel: w364 -> [w386 _]
              tunnel: ["UpdateWirePreView\nUpdate" _] -> w362
              frame 0, Default {
                w370 = T4 {"Decal"=FALSE, "Color"=11184810} ("Edge color")
                n237 = Index Array(array=w386, index=w385) -> (element=w369:T8)
                n238 = Unbundle By Name(w369) -> ("Edge thickness"=w372:i32, "Edge color"=w384:u32, "Center thickness"=w375:i32, "Center pattern"=w376:T5, "CenterColor1"=w383:u32, "CenterColor2"=w382:u32, "Tunnels and terminals colors"=w381:u32)
                n239 = Decrement(x=w375) -> (x-1=w374:i32)
                n240 = Bundle(cluster=w370, "Color"=w384) -> (w377:T4)  [unwired: 1 in]
                n241 = Bundle(cluster=w370, "Color"=w383) -> (w378:T4)  [unwired: 1 in]
                n242 = Bundle(cluster=w370, "Color"=w382) -> (w379:T4)  [unwired: 1 in]
                n243 = Bundle(cluster=w370, "Color"=w381) -> (w380:T4)  [unwired: 1 in]
                n244 = local write "_TunnelsAndTerminalsColors"(w380) -> ()
                n245 = To Unsigned Word Integer(number=w372) -> (unsigned 16bit integer=w371:u16)
                n246 = To Unsigned Word Integer(number=w374) -> (unsigned 16bit integer=w373:u16)
                n247 = local write "_CenterThickness"(w373) -> ()
                n248 = local write "_EdgeThickness"(w371) -> ()
                n249 = local write "_CenterPattern"(w376) -> ()
                n250 = local write "_CenterColor1"(w378) -> ()
                n251 = local write "_CenterColor2"(w379) -> ()
                n252 = local write "_EdgeColor"(w377) -> ()
              }
              frame -1 {
              }
            }
          }
          event "DeleteWireStyle": Value Change {
            n253 = event-data() -> ()  [unwired: 1 in, 6 out]
            n254 = local read "WireStyleList"() -> (w390:T2[])
            n255 = for {
              tunnel: w390 -> [w397] mode=indexing
              tunnel: [w395] -> w389
              tunnel: [w394] -> _
              tunnel: [w393] -> w388
              i -> [w394]
              stop <- w393 stop-if-true
              n256 = Unbundle By Name(w397) -> ("Name"=w395:string, "Status"=w396:u16)
              n257 = Not Equal To 0?(x=w396) -> (x != 0?=w393:bool)
            }
            n258 = case shown="True" w388 {
              tunnel: w389 -> [_ w391]
              frame False {
              }
              frame True {
                n259 = call "BaseProvider_WireStylesManager.vi"("Action(Read)"=enum16{"Read", "UpdateOne", "DeleteOne"}."DeleteOne", "WireStyleName(Default)"=w391) -> ()  [unwired: 6 in, 4 out]
              }
            }
          }
          event "Update/AddWireStyle": Value Change {
            n260 = event-data() -> ()  [unwired: 1 in, 6 out]
            n261 = Unbundle By Name(w402) -> ("CurrentWireStyle"=w401:T8)
            n262 = local read "WireStyleName"() -> (w399:string)
            n263 = call "BaseProvider_WireStylesManager.vi"("Action(Read)"=enum16{"Read", "UpdateOne", "DeleteOne"}."UpdateOne", "WireConfiguration(New or Updating)"=w401, "WireStyleName(Default)"=w399) -> ()  [unwired: 5 in, 4 out]
          }
          event "Up", "Down": Value Change {
            n264 = event-data() -> ()  [unwired: 1 in, 6 out]
            n265 = local read "WireStyleList"() -> (w413:T2[])
            n266 = Unbundle By Name(w416) -> ("CurrentWireStyle"=w415:T8)
            n267 = for {
              tunnel: w413 -> [w421] mode=indexing
              tunnel: [w418] -> w404
              tunnel: [w417] -> w411
              i -> [w417]
              stop <- w419 stop-if-true
              n268 = Unbundle By Name(w421) -> ("Name"=w418:string, "Status"=w420:u16)
              n269 = Not Equal To 0?(x=w420) -> (x != 0?=w419:bool)
            }
            n270 = Increment(x=w411) -> (x+1=w412:i32)
            n271 = Decrement(x=w411) -> (x-1=w410:i32)
            n272 = Select(t=w412, s="Down", f=w410) -> (s? t:f=w406:i32)
            n273 = call "BaseProvider_WireStylesManager.vi"("Action(Read)"=enum16{"Read", "UpdateOne", "DeleteOne"}."UpdateOne", "NewIndex(-1=NoChange/Inserted Last If not found)"=w406, "WireConfiguration(New or Updating)"=w415, "WireStyleName(Default)"=w404) -> ("AllWireConfigurations(Names)"=w405:string[])  [unwired: 4 in, 3 out]
            n274 = Search 1D Array(1D array=w405, element=w404) -> (index of element=w403:i32)  [unwired: 1 in]
            n275 = Format Into String(format string="UpdateWirePreView\nUpdateWireStyleList>>%d\nUpdate", w403) -> (resulting string=w407:string)  [unwired: 2 in, 1 out]
          }
          event "_Dice": Mouse Enter {
            n276 = event-data() -> ()  [unwired: 1 in, 1 out]
            n277 = local write "_Dice"(cluster{"Boolean 2":bool, "Dice":bool} {"Boolean 2"=TRUE, "Dice"=FALSE} ("Dice")) -> ()
          }
          event "_Dice": Mouse Leave {
            n278 = event-data() -> ()  [unwired: 1 in, 1 out]
            n279 = local write "_Dice"(cluster{"Boolean 2":bool, "Dice":bool} {"Boolean 2"=FALSE, "Dice"=FALSE} ("Dice")) -> ()
          }
          event "_HelpDefaultConfiguration": Value Change {
            n280 = event-data() -> ()  [unwired: 1 in, 1 out]
            n281 = fn#1354() -> (1:w427:bool)  [unwired: 1 out]
            n282 = Not(x=w427) -> (.not. x?=w426:bool)
            n283 = Control Help Window(1:w426) -> ()  [unwired: 1 in]
          }
        }
      }
      frame "UpdateClass" {
        n284 = local read "_CenterColor1"() -> (w450:T4)
        n285 = local read "_CenterColor2"() -> (w454:T4)
        n286 = local read "_EdgeColor"() -> (w452:T4)
        n287 = local read "_EdgeThickness"() -> (w456:T7)
        n288 = local read "_CenterThickness"() -> (w451:T6)
        n289 = local read "_TunnelsAndTerminalsColors"() -> (w449:T4)
        n290 = local read "_CenterPattern"() -> (w459:T5)
        n291 = Format Into String("_DefaultConnectorPanePattern") -> (resulting string=w432:string)  [unwired: 3 in, 1 out]
        n292 = Unbundle By Name(w464) -> ("ClassRefCreated"=w466:bool, "ClassRef"=w431:refnum<vi>)
        n293 = disable-structure shown="Enabled" {
          disable-tunnel: [w475 _] -> w444
          frame Enabled {
            n294 = property on="_Icon" class="Ring (strict)"() -> ("Strings []"=w477:string[])  [unwired: 2 in, 2 out]
            n295 = local read "_Icon"() -> (w476:u16)
            n296 = Index Array(array=w477, index=w476) -> (element=w475:string)
          }
          frame Disabled {
          }
        }
        n297 = To Unsigned Long Integer(number=w451) -> (unsigned 32bit integer=w453:u32)
        n298 = Unbundle(w450) -> ("Color"=w460:u32)  [unwired: 1 out]
        n299 = Unbundle(w454) -> ("Color"=w461:u32)  [unwired: 1 out]
        n300 = Unbundle(w449) -> ("Color"=w462:u32)  [unwired: 1 out]
        n301 = Unbundle(w452) -> ("Color"=w457:u32)  [unwired: 1 out]
        n302 = Increment(x=w453) -> (x+1=w458:u32)
        n303 = call "GDSLvClass_ReadClassType.vi"("Class Refnum In"=w431, "error in (no error)"=w436) -> ("Class Refnum Out"=w438:refnum<vi>, "ClassSettings"=w435:T13, "error out"=w439:errorcluster)  [unwired: 15 in]
        n304 = Bundle By Name(cluster=w435, "ConnectorPanePattern"=w432) -> (w434:T13)
        n305 = call "GDSLvClass_StoreClassType.vi"("Class Refnum In"=w438, "ClassSettings"=w434, "error in (no error)"=w439) -> ("Class Refnum Out"=w430:refnum<vi>, "error out"=w437:errorcluster)  [unwired: 15 in]
        n306 = Bundle(cluster=T8 {"Edge thickness"=0, "Edge color"=0, "Center thickness"=0, "Center pattern"=enum."Solid", "CenterColor1"=0, "CenterColor2"=0, "Tunnels and terminals colors"=0} ("WireConfiguration"), "Edge thickness"=w456, "Edge color"=w457, "Center thickness"=w458, "Center pattern"=w459, "CenterColor1"=w460, "CenterColor2"=w461, "Tunnels and terminals colors"=w462) -> (w448:T8)
        n307 = disable-structure shown="Enabled" {
          disable-tunnel: w444 -> [w473 _]
          disable-tunnel: [w470 w474] -> w429
          disable-tunnel: w437 -> [w472 w474]
          disable-tunnel: w430 -> [w471 _]
          frame Enabled {
            n308 = call "GDSLvClass_StoreClassItemIcon.vi"("Library Refnum"=w471, "ClassItemIconName"=w473, "error in (no error)"=w472) -> ("error out"=w470:errorcluster)  [unwired: 15 in, 1 out]
          }
          frame Disabled {
          }
        }
        n309 = call "GOOP_WirePenTranslator.vi"("WireConfigurationIn"=w448) -> ("WirePensOut"=w463:T16)  [unwired: 17 in, 1 out]
        n310 = property class="LVClassLibrary"(reference=w430, error in=w429, "Wire Pens"=w463) -> (reference out=w447:refnum<vi>, error out=w446:errorcluster)
        n311 = invoke class="LVClassLibrary" method="Save"(reference=w447, error in=w446) -> (reference out=w445:refnum<vi>, error out=w441:errorcluster)  [unwired: 2 in, 2 out]
        n312 = case shown="True" w466 {
          tunnel: w441 -> [w481 w484]
          tunnel: w445 -> [_ w483]
          tunnel: [w481 w482] -> w440
          frame False {
          }
          frame True {
            n313 = Close Reference(reference=w483, error in (no error)=w484) -> (error out=w482:errorcluster)
          }
        }
        n314 = Unbundle By Name(w440) -> ("code"=w443:i32)
        n315 = case shown="Default" w443 {
          tunnel: w436 -> [w478 _]
          tunnel: [w478 w480] -> w442
          tunnel: w440 -> [_ w480]
          frame 8 {
            n316 = One Button Dialog(message="Warning\nThe changes could not be saved.\nThe file might be read-only.") -> ()  [unwired: 1 in, 1 out]
          }
          frame Default {
          }
        }
        n317 = Select(t="SaveConfiguration", s="_SetToDefaultForAllClasses", f="Exit") -> (s? t:f=w469:string)
      }
      frame "UpdateIconPreview" {
        n318 = property on="_Icon" class="Ring (strict)"() -> ("Strings []"=w488:string[])  [unwired: 2 in, 2 out]
        n319 = local read "_Icon"() -> (w487:u16)
        n320 = Index Array(array=w488, index=w487) -> (element=w486:string)
        n321 = call "GOOP_GetOverlayIconPath.vi"("IconName(NoPngExtension)"=w486) -> ("IconPath"=w485:path)  [unwired: 10 in]
        n322 = Empty String/Path?(string/path=w485) -> (empty?=w489:bool)
        n323 = case shown="False" w489 {
          tunnel: w485 -> [w493 _]
          frame False {
            n324 = call <vilib>:"Read PNG File.vi"("path to PNG file"=w493) -> ("image data"=w496:T18)  [unwired: 8 in, 2 out]
            n325 = call "GOOP_DrawWirePreview_ZoomImage.vi"("image data 2"=w496, "Zoom"=5) -> ("image data"=w497:T18)
            n326 = call <vilib>:"Draw Flattened Pixmap.vi"("image data"=w497) -> ("new picture"=→"_Preview":picture)  [unwired: 8 in]
          }
          frame True {
          }
        }
      }
      frame "SaveConfiguration" {
        n327 = local read "_CenterColor1"() -> (w518:T4)
        n328 = local read "_CenterColor2"() -> (w517:T4)
        n329 = local read "_EdgeColor"() -> (w521:T4)
        n330 = local read "_EdgeThickness"() -> (w522:T7)
        n331 = local read "_CenterThickness"() -> (w520:T6)
        n332 = local read "_TunnelsAndTerminalsColors"() -> (w516:T4)
        n333 = local read "_CenterPattern"() -> (w519:T5)
        n334 = local read "_DefaultConnectorPanePattern"() -> (w511:T3)
        n335 = property on="_Icon" class="Ring (strict)"() -> ("Strings []"=w508:string[])  [unwired: 2 in, 2 out]
        n336 = local read "_Icon"() -> (w509:u16)
        n337 = Index Array(array=w508, index=w509) -> (element=w507:string)
        n338 = To Unsigned Long Integer(number=w520) -> (unsigned 32bit integer=w529:u32)
        n339 = case shown="True" w510 {
          tunnel: [w530 w536] -> w506
          tunnel: w507 -> [w530 w531]
          frame False {
          }
          frame True {
            n340 = call "BaseProvider_IniFileSettings.vi"() -> ("IniFileSettings"=w534:T12, "error out"=w532:errorcluster)  [unwired: 18 in]
            n341 = Bundle By Name(cluster=w534, "InterfaceIcon"=w531) -> (w535:T12)
            n342 = call "BaseProvider_ConfigurationMemory.vi"() -> ("IconOut"=w536:string)  [unwired: 13 in, 6 out]
            n343 = call "BaseProvider_IniFileSettings.vi"("IniFileSettings"=w535, "error in (no error)"=w532, "Action"=enum16{"Read", "Load", "Save"}."Save") -> ()  [unwired: 15 in, 2 out]
          }
        }
        n344 = Increment(x=w529) -> (x+1=w528:u32)
        n345 = Unbundle(w518) -> ("Color"=w526:u32)  [unwired: 1 out]
        n346 = Unbundle(w517) -> ("Color"=w527:u32)  [unwired: 1 out]
        n347 = Unbundle(w516) -> ("Color"=w524:u32)  [unwired: 1 out]
        n348 = Unbundle(w521) -> ("Color"=w525:u32)  [unwired: 1 out]
        n349 = Bundle By Name(cluster=T8 {"Edge thickness"=0, "Edge color"=0, "Center thickness"=0, "Center pattern"=enum."Solid", "CenterColor1"=0, "CenterColor2"=0, "Tunnels and terminals colors"=0} ("WireConfiguration"), "Edge thickness"=w522, "Edge color"=w525, "Center thickness"=w528, "Center pattern"=w519, "CenterColor1"=w526, "CenterColor2"=w527, "Tunnels and terminals colors"=w524) -> (w500:T8)
        n350 = call "BaseProvider_WireStylesManager.vi"() -> ("AllWireConfigurations"=w501:T8[])  [unwired: 8 in, 3 out]
        n351 = call "BaseProvider_ConfigurationMemory.vi"("WireConfiguration"=w500, "Icon"=w506, "Action"=enum16{"Read", "Load", "Save"}."Save", "PatternIn"=w511) -> ()  [unwired: 9 in, 7 out]
        n352 = Bundle By Name(cluster=T10 {"FlatFolderStructure"=FALSE} ("OptionsIn"), "FlatFolderStructure"="_FlatFolderStructure") -> (w505:T10)
        n353 = Search 1D Array(1D array=w501, element=w500) -> (index of element=w498:i32)  [unwired: 1 in]
        n354 = Bundle By Name(cluster=w513, "SelectedWireStyleIndex"=w498) -> (w499:T9)
        n355 = call "GOOP400_ConfigurationMemory.vi"("OptionsIn"=w505, "Action"=enum16{"Read", "Load", "Save"}."Save") -> ()  [unwired: 16 in, 2 out]
      }
    }
  }
  "Error Out" <- w27
  n356 = disable-structure shown="Disabled" {
    frame Disabled {
      n357 = property on="_EdgeThickness" class="Enum (strict)"("Val(Sgnl)"=T7."1 pixel" ("Value (Signaling)")) -> ()  [unwired: 2 in, 2 out]
    }
    frame Enabled {
    }
  }
  n358 = Generate User Event(user event=w25, event data cluster="Stop" ("Stop")) -> (user event out=w26:refnum<user-event>)  [unwired: 2 in, 1 out]
  n359 = Destroy User Event(user event=w26) -> (error out=w14:errorcluster)  [unwired: 1 in]
  n360 = Destroy User Event(user event=w12, error in=w14) -> (error out=w13:errorcluster)
  n361 = case shown="False" w11 {
    tunnel: [CommonVIs_ClassIconSelection_Action."All" ("IconsToShow(All)") CommonVIs_ClassIconSelection_Action."Only Interface" ("IconsToShow(All)")] -> w4
    frame False {
    }
    frame True {
    }
  }
  n362 = Unregister For Events(event registration refnum=w15, error in=w13) -> ()  [unwired: 1 out]
  n363 = control-ref of="IconSelection"() -> (w2:refnum<vi>)
  n364 = control-ref of="Icon"() -> (w3:refnum<vi>)
  n365 = call "CommonVIs_ClassIconSelection.vi"("SaveChangesInClassRightAway(True)"=FALSE, "IconSelected"=w12, "IconsToShow(All)"=w4, "Icon"=w3, "error in (no error)"=w10, "Messages(Stop or Empty string will stop this VI)"=w20, "IconSelection"=w2, "LVClassToActOn"=w17) -> ()  [unwired: 4 in]
  n366 = call "GDSString_AddStatesToQueue.vi"() -> ()  [unwired: 15 in, 1 out]
  n367 = Unbundle By Name(w6) -> ("SelectedWireStyleIndex"=→"SelectedWireStyleIndex":i32)
